vi "SPARK Configure Encoder.vi"   [LabVIEW 2023]
doc: "Configure the primary encoder of the SPARK."
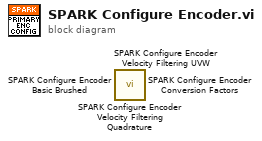
[diagram p0: block diagram]
diagram:
  n1 = call <vilib>:"SPARK Configure Encoder Velocity Filtering Quadrature.vi"() -> ()  [unwired: 10 in, 2 out]
  n2 = call <vilib>:"SPARK Configure Encoder Velocity Filtering UVW.vi"() -> ()  [unwired: 10 in, 2 out]
  n3 = call <vilib>:"SPARK Configure Encoder Basic Brushed.vi"() -> ()  [unwired: 10 in, 2 out]
  n4 = call <vilib>:"SPARK Configure Encoder Conversion Factors.vi"() -> ()  [unwired: 10 in, 2 out]
